vi "Create CIF PCAP DAQ Config.vi"(9 "Custom Data":u8[](array[numeric]) format="%.0x", 10 "Max Msg/FIFO":u64=5, 11 "DAQ FIFO Config":T1={"Max Samples"=100000, "Max Channels"=1, "FIFO Flags"={"Backpressure"=FALSE}, "Best Effort Subscribers"=2, "Backpressure Subscribers"=0}) -> (3 "Flattened FIFO Config":u8[](array[numeric]))   [LabVIEW 2021, in "Iceoryx Channel Utilities.lvlib"]
uses:
  Iceoryx Channel Utilities.lvlib
  Typedef/DAQ FIFO Config.ctl
  ChannelCommon/typedef/New FIFO Config.ctl
  ChannelCommon/typedef/FIFO Flags.ctl
  ChannelCommon/ChannelCommon.lvlib
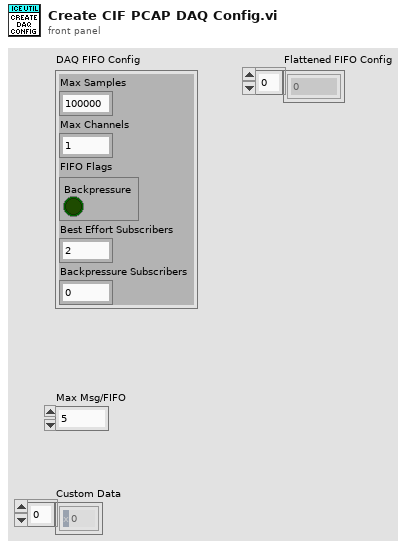
[diagram p1: front panel]
types:
  T1 = typedef "Iceoryx Channel Utilities.lvlib/DAQ FIFO Config.ctl" = cluster{"Max Samples":u64, "Max Channels":u64, "FIFO Flags":cluster{"Backpressure":bool}, "Best Effort Subscribers":u32, "Backpressure Subscribers":u32}
  T2 = typedef "ChannelCommon.lvlib/New FIFO Config.ctl" = cluster{"Max Bytes/Msg":u64, "Max Msg/FIFO":u64, "FIFO Flags":T3, "Best Effort Subscribers":u32, "Backpressure Subscribers":u32}
  T3 = typedef "ChannelCommon.lvlib/FIFO Flags.ctl" = cluster{"Backpressure":bool, "Extended Config":bool}
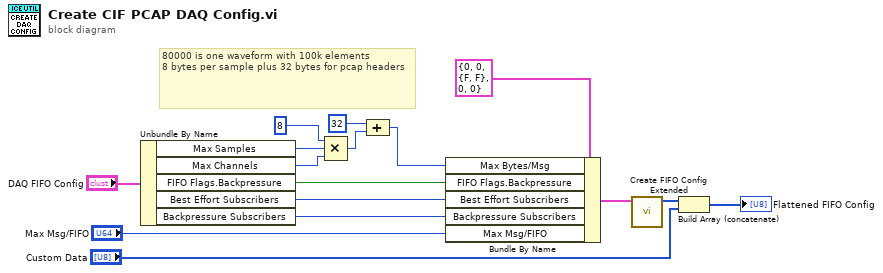
[diagram p0: block diagram]
diagram:
  # "80000 is one waveform with 100k elements\n8 bytes per sample plus 32 bytes for pcap headers"
  n1 = Unbundle By Name("DAQ FIFO Config") -> ("Max Samples"=w13:u64, "Max Channels"=w14:u64, "FIFO Flags.Backpressure"=w1:bool, "Best Effort Subscribers"=w8:u32, "Backpressure Subscribers"=w6:u32)
  n2 = Compound Arithmetic op=MULTIPLY(u64 8 ("value"), w13, w14) -> (w12:u64)
  n3 = Compound Arithmetic op=ADD(u64 32 ("value"), w12) -> (w11:u64)
  n4 = Bundle By Name(cluster=T2 {"Max Bytes/Msg"=0, "Max Msg/FIFO"=0, "FIFO Flags"={"Backpressure"=FALSE, "Extended Config"=FALSE}, "Best Effort Subscribers"=0, "Backpressure Subscribers"=0} ("New FIFO Config"), "Max Bytes/Msg"=w11, "FIFO Flags.Backpressure"=w1, "Best Effort Subscribers"=w8, "Backpressure Subscribers"=w6, "Max Msg/FIFO"="Max Msg/FIFO") -> (w5:T2)
  n5 = call "Create FIFO Config Extended.vi"("New FIFO Config"=w5) -> ("Flattened FIFO Config"=w4:u8[])  [unwired: 10 in]
  n6 = Build Array (concatenate)(w4, "Custom Data") -> (→"Flattened FIFO Config":u8[])
